vi "get Marker Value.vi"(8 "error in (no error)":errorcluster, 10 "Marker Index":i32, 11 "SA Measurement in":refnum<class "SA Measurement.lvclass">) -> (0 "error out":errorcluster, 2 "Marker Value":T1, 3 "SA Measurement out":refnum<class "SA Measurement.lvclass">)   [LabVIEW 2023, in "Spectrum Analyzer.lvlib" / "SA Measurement.lvclass"]
uses:
  SA Measurement.lvclass
  SA Measurement.lvclass/SA Measurement.ctl
  Interface_Spectrum/Interface_Spectrum.lvclass
  TYPE DEFINITION/TYPE Marker Control Mode.ctl
  Spectrum Analyzer.lvlib
panel:
  in  "Trace Index":i32
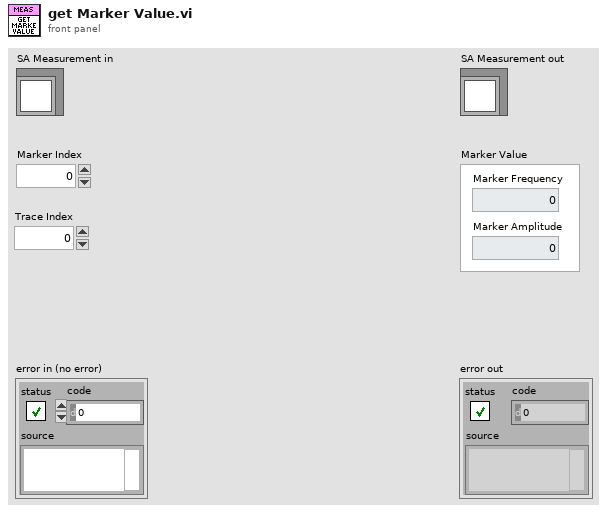
[diagram p1: front panel]
types:
  T1 = cluster{"Marker Frequency":dbl, "Marker Amplitude":dbl}
  T2 = typedef "Spectrum Analyzer.lvlib/TYPE Marker Control Mode.ctl" = enum16{"Normal", "Delta", "Off"}
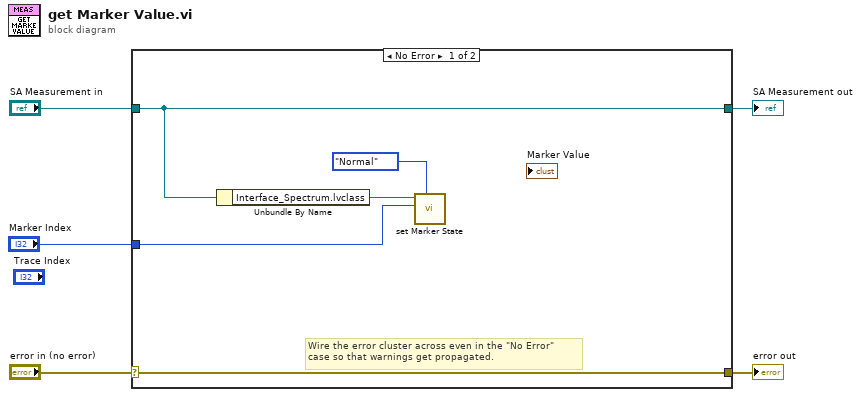
[diagram p0: block diagram]
diagram:
  n1 = case shown="No Error" "error in (no error)" {
    selector: "error in (no error)" -> [w10 w12]
    tunnel: [w10 w12] -> w4
    tunnel: [w9 w11] -> w2
    tunnel: "SA Measurement in" -> [w9 w11]
    tunnel: "Marker Index" -> [w6 _]
    frame No Error {
      # "Wire the error cluster across even in the \"No Error\"\ncase so that warnings get propagated."
      n2 = Unbundle By Name(w9) -> ("Interface_Spectrum.lvclass"=w7:refnum<class "Interface_Spectrum.lvclass">)
      n3 = call-dynamic "set Marker State.vi"("Marker Mode"=TYPE_Marker_Control_Mode."Normal", "Marker Index"=w6, "Interface_Spectrum in"=w7) -> ()  [unwired: 7 in, 2 out]
    }
    frame Error {
    }
  }
  "error out" <- w4
  "SA Measurement out" <- w2
